vi "RemoteVI List Menus.vi"() -> (4 "menus":T1(array[cluster]))   [LabVIEW 2020, in "RemoteVI.lvlib"]
doc: "Lists the visible LabVIEW menu windows (class LVMenuWnd - ring and enum menus, shortcut menus, their submenus, and custom popups such as the colour picker and the line width popup of a plot legend) top-most first, each with its screen rectangle. A submenu is shown above its parent, so menus[0] is the deepest open menu and the menu a key goes to. Walks the top-level LVMenuWnd windows with user32 FindWindowExW(0, previous, \"LVMenuWnd\", NULL) in z-order, keeps the visible ones (user32 IsWindowVisible) and reads their rectangle (user32 GetWindowRect). Cheap, no full window walk (RemoteVI Find Popups.vi takes about 30 ms). LabVIEW's menus are never moved by the server any more, so these real rectangles are also the logical ones. Errors of the calls end the walk and are dropped; a window that closes meanwhile is simply missing. Win32 only, no VI Server call, so it runs while an open menu holds LabVIEW's UI thread."
uses:
  RemoteVI.lvlib
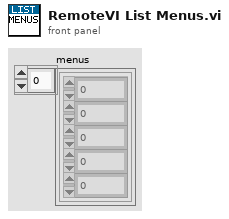
[diagram p1: front panel]
types:
  T1 = cluster{"hwnd":u64, "x":i32, "y":i32, "w":i32, "h":i32}[]
  T2 = cluster{"hwnd":u64, "x":i32, "y":i32, "w":i32, "h":i32}
  T3 = cluster{"left":i32, "top":i32, "right":i32, "bottom":i32}
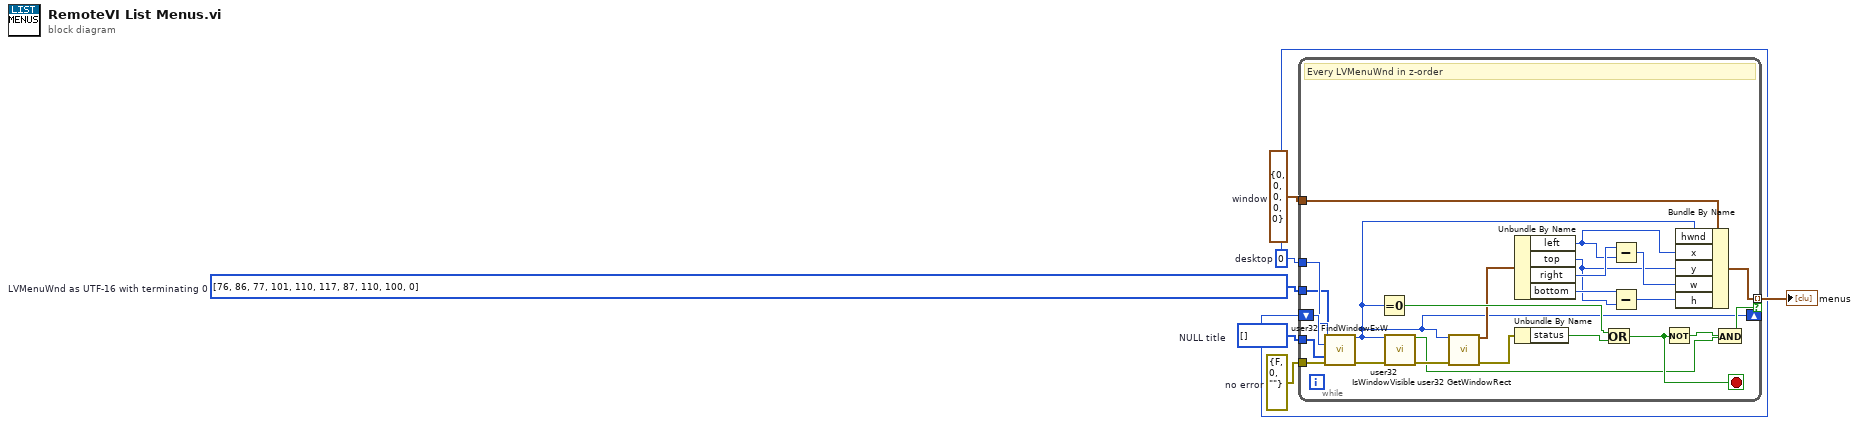
[diagram p0: block diagram]
diagram:
  w5 = errorcluster {"status"=FALSE, "code"=0, "source"=""}  # no error
  w4 = T2 {"hwnd"=0, "x"=0, "y"=0, "w"=0, "h"=0}  # window
  w3 = u64 0  # desktop
  w2 = u16[] []  # NULL title
  w1 = u16[] [76, 86, 77, 101, 110, 117, 87, 110, 100, 0]  # LVMenuWnd as UTF-16 with terminating 0
  n1 = while {
    tunnel: w1 -> [w7]
    tunnel: w2 -> [w8]
    tunnel: w3 -> [w9]
    tunnel: w4 -> [w10]
    tunnel: w5 -> [w11]
    shift-right: [w13] -> _
    shift-left: w3 -> [w12]
    tunnel: [w25] -> w6 mode=indexing if=w30
    stop <- w28 stop-if-true
    # "Every LVMenuWnd in z-order"
    n2 = call "user32 FindWindowExW.vi"("hWndParent"=w9, "hWndChildAfter"=w12, "lpszClass"=w7, "lpszWindow"=w8, "error in"=w11) -> ("hWnd"=w13:u64, "error out"=w14:errorcluster)  [unwired: 9 in]
    n3 = Equal To 0?(x=w13) -> (x = 0?=w26:bool)
    n4 = call "user32 IsWindowVisible.vi"("hWnd"=w13, "error in"=w14) -> ("visible?"=w15:bool, "error out"=w16:errorcluster)  [unwired: 12 in]
    n5 = call "user32 GetWindowRect.vi"("hWnd"=w13, "error in"=w16) -> ("RECT"=w17:T3, "error out"=w18:errorcluster)  [unwired: 11 in, 1 out]
    n6 = Unbundle By Name(w17) -> ("left"=w19:i32, "top"=w20:i32, "right"=w21:i32, "bottom"=w22:i32)
    n7 = Unbundle By Name(w18) -> ("status"=w27:bool)
    n8 = Or(x=w26, y=w27) -> (x .or. y?=w28:bool)
    n9 = Subtract(x=w21, y=w19) -> (x-y=w23:i32)
    n10 = Subtract(x=w22, y=w20) -> (x-y=w24:i32)
    n11 = Not(x=w28) -> (.not. x?=w29:bool)
    n12 = Bundle By Name(cluster=w10, "hwnd"=w13, "x"=w19, "y"=w20, "w"=w23, "h"=w24) -> (w25:T2)
    n13 = And(x=w29, y=w15) -> (x .and. y?=w30:bool)
  }
  "menus" <- w6
